vi "ADT681_Read.vi"(7 "Error In":errorcluster, 10 "DriverConnect in":T1={"InterfaceType"=enum."VISA", "OpenedSession"="COM4", "InterfaceSettings"={"Interface"=enum."RS232", "EOS 4 read"=enum."Default (=EOS 4 write)", "EOS 4 write"=enum."CR (\\r)", "TMO, ms"=2000, "Sett"=variant(cluster{"Baud Rate":u32, "Data Bits":u16, "Parity":u16, "Stop Bits":u16, "Flow Control":u16, "Eho":bool} {"Baud Rate"=75, "Data Bits"=0, "Parity"=0, "Stop Bits"=0, "Flow Control"=0, "Eho"=FALSE})}}) -> (0 "Error Out":errorcluster, 3 "DriverConnect out":T1={"InterfaceType"=enum."VISA", "OpenedSession"="COM4", "InterfaceSettings"={"Interface"=enum."RS232", "EOS 4 read"=enum."Default (=EOS 4 write)", "EOS 4 write"=enum."CR (\\r)", "TMO, ms"=2000, "Sett"=variant(cluster{"Baud Rate":u32, "Data Bits":u16, "Parity":u16, "Stop Bits":u16, "Flow Control":u16, "Eho":bool} {"Baud Rate"=75, "Data Bits"=0, "Parity"=0, "Stop Bits"=0, "Flow Control"=0, "Eho"=FALSE})}}, 4 "String":string)   [LabVIEW 2018]
uses:
  MOKO_LabViewLibrary/MokoLowLevel/MokoLowLovelControl/MLLC_ConnectCluster.ctl
  MOKO_LabViewLibrary/MokoLowLevel/MokoLowLovelControl/MLLC_InterfaceType.ctl
  MOKO_LabViewLibrary/MokoLowLevel/MokoLowLovelControl/MLLC_OpenedSession.ctl
  MOKO_LabViewLibrary/MokoLowLevel/MokoLowLovelControl/MLLC_InterfaceSettings.ctl
  MOKO_LabViewLibrary/MokoLowLevel/MokoLowLovelControl/MLLC_InterfaceKind.ctl
panel:
  out "read buffer":string
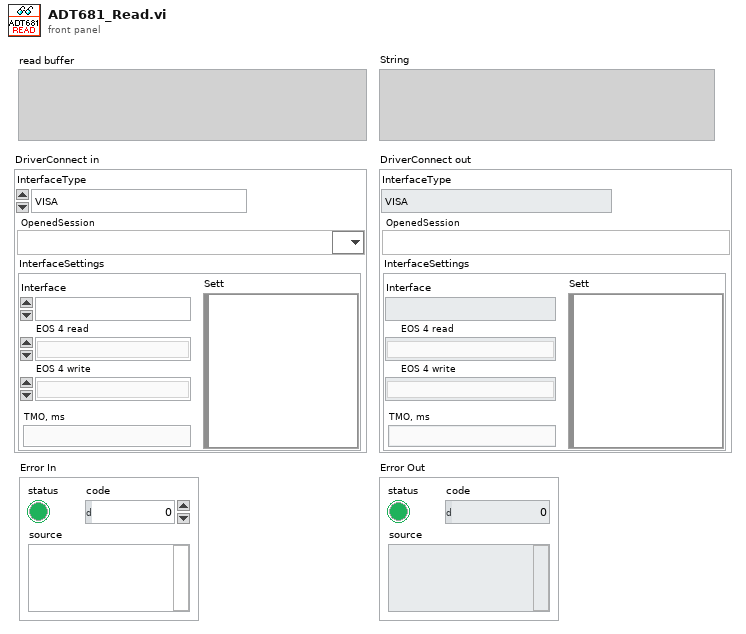
[diagram p1: front panel]
types:
  T1 = typedef "MLLC_ConnectCluster.ctl" = cluster{"InterfaceType":T2, "OpenedSession":T3, "InterfaceSettings":T4}
  T2 = typedef "MLLC_InterfaceType.ctl" = enum16{"VISA", "Prologix USB-GPIB"}
  T3 = typedef "MLLC_OpenedSession.ctl" = refnum<visa-resource-name>
  T4 = typedef "MLLC_InterfaceSettings.ctl" = cluster{"Interface":T5, "EOS 4 read":enum16{"Default (=EOS 4 write)", "CR (\\r)", "LF (\\n)", "None"}, "EOS 4 write":enum16{"CR+LF (\\r\\n)", "CR (\\r)", "LF (\\n)", "None"}, "TMO, ms":i32, "Sett":variant}
  T5 = typedef "MLLC_InterfaceKind.ctl" = enum16{"RS232", "GPIB", "USB", "Ethernet", "another"}
  T6 = enum16{"Default (=EOS 4 write)", "CR (\\r)", "LF (\\n)", "None"}
  T7 = enum16{"CR+LF (\\r\\n)", "CR (\\r)", "LF (\\n)", "None"}
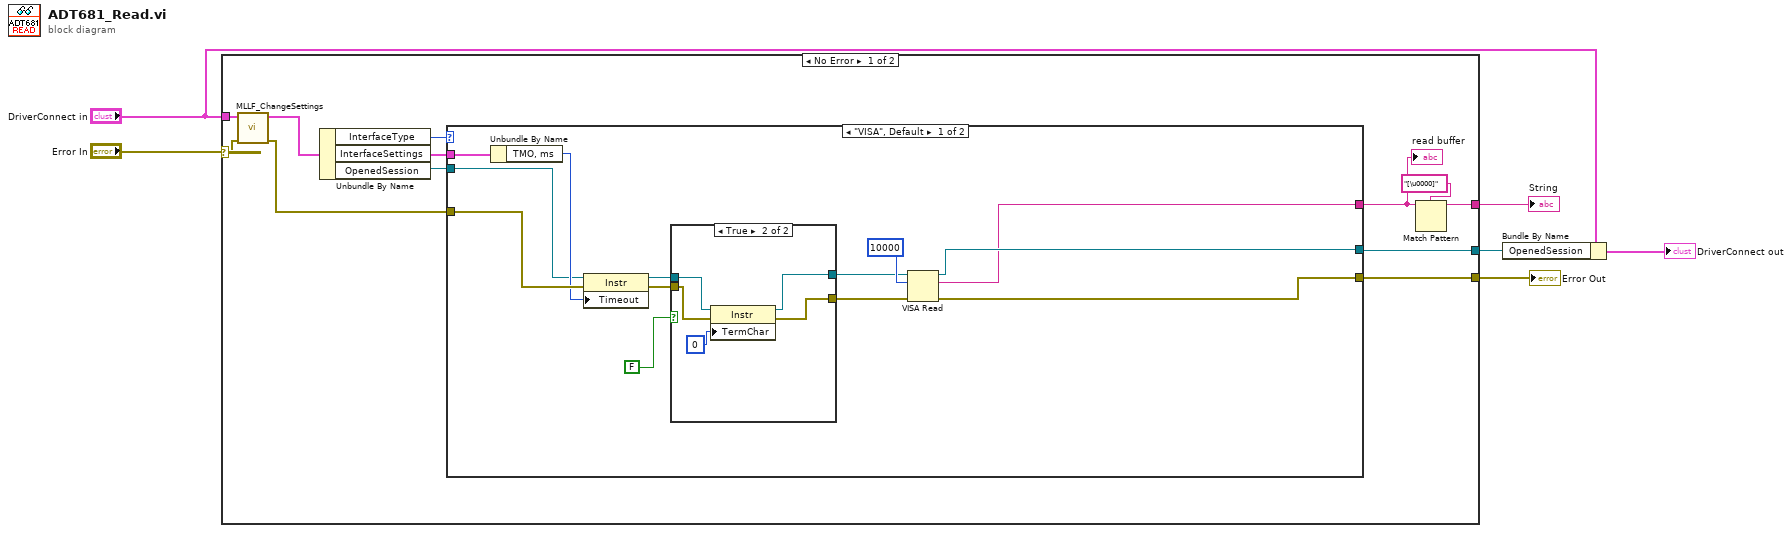
[diagram p0: block diagram]
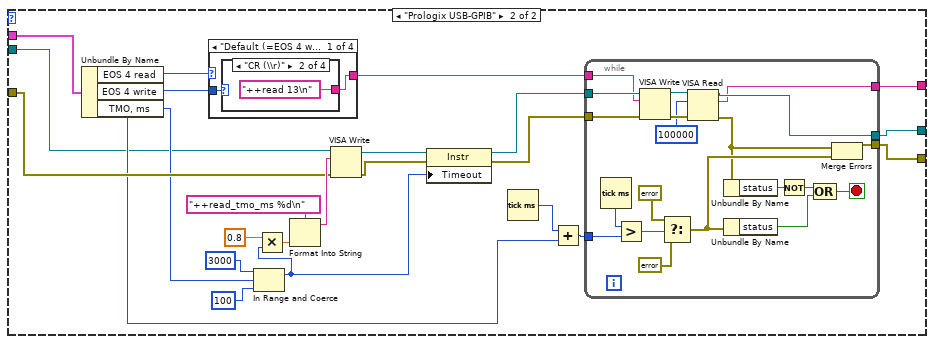
[diagram p3: hidden frame]
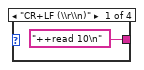
[diagram p4: hidden frame]
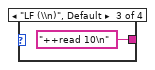
[diagram p5: hidden frame]
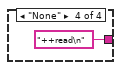
[diagram p6: hidden frame]
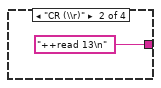
[diagram p7: hidden frame]
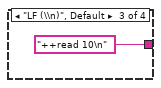
[diagram p8: hidden frame]
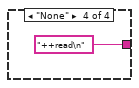
[diagram p9: hidden frame]
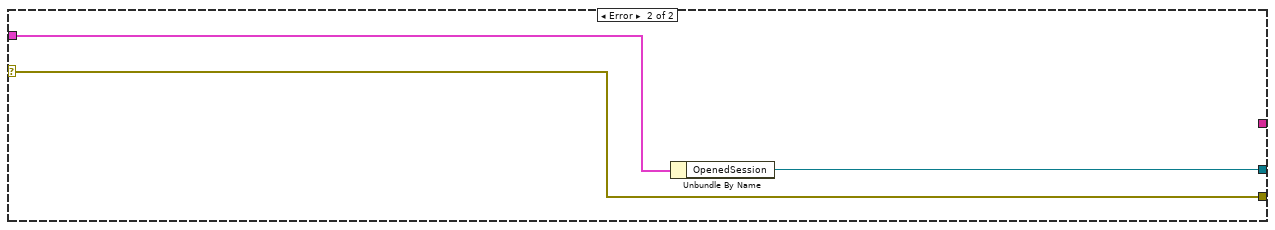
[diagram p10: hidden frame]
diagram:
  n1 = case shown="No Error" "Error In" {
    selector: "Error In" -> [w15 w93]
    tunnel: [w18 _] -> w6
    tunnel: [w17 w93] -> w4
    tunnel: [w16 w91] -> w2
    tunnel: "DriverConnect in" -> [w11 w92]
    frame No Error {
      n2 = call "MLLF_ChangeSettings.vi"("Error In"=w15, "DriverConnect in"=w11) -> ("Error Out"=w13:errorcluster, "DriverConnect out"=w10:T1)  [unwired: 4 in]
      n3 = Unbundle By Name(w10) -> ("InterfaceType"=w9:T2, "InterfaceSettings"=w8:T4, "OpenedSession"=w7:T3)
      n4 = case shown="\"VISA\", Default" w9 {
        tunnel: [w31 w44] -> w17
        tunnel: [w30 w43] -> w16
        tunnel: [w29 w61] -> w12
        tunnel: w13 -> [w28 w42]
        tunnel: w8 -> [w20 w60]
        tunnel: w7 -> [w19 w39]
        frame "VISA", Default {
          n5 = Unbundle By Name(w20) -> ("TMO, ms"=w27:i32)
          n6 = property class="Instr"(reference=w19, error in=w28, "Timeout"=w27) -> (reference out=w25:T3, error out=w24:errorcluster)
          n7 = case shown="True" FALSE {
            tunnel: w25 -> [w33 w37]
            tunnel: w24 -> [w32 w36]
            tunnel: [w33 w35] -> w23
            tunnel: [w32 w34] -> w22
            frame False {
            }
            frame True {
              n8 = property class="Instr"(reference=w37, error in=w36, "TermChar"=u8 0 ("Message Based Settings:Termination Character")) -> (reference out=w35:T3, error out=w34:errorcluster)
            }
          }
          n9 = VISA Read(VISA resource name=w23, byte count=u32 10000, error in (no error)=w22) -> (VISA resource name out=w30:T3, read buffer=w29:string, error out=w31:errorcluster)  [unwired: 1 out]
        }
        frame "Prologix USB-GPIB" {
          n10 = Unbundle By Name(w60) -> ("EOS 4 read"=w47:T6, "EOS 4 write"=w45:T7, "TMO, ms"=w41:i32)
          n11 = case shown="\"Default (=EOS 4 write)\"" w47 {
            tunnel: [w62 "++read 13\n" ("write buffer") "++read 10\n" ("write buffer") "++read\n" ("write buffer")] -> w46
            tunnel: w45 -> [w63 _ _ _]
            frame "Default (=EOS 4 write)" {
              n12 = case shown="\"CR (\\\\r)\"" w63 {
                tunnel: ["++read 10\n" ("write buffer") "++read 13\n" ("write buffer") "++read 10\n" ("write buffer") "++read\n" ("write buffer")] -> w62
                frame "CR+LF (\\r\\n)" {
                }
                frame "CR (\\r)" {
                }
                frame "LF (\\n)", Default {
                }
                frame "None" {
                }
              }
            }
            frame "CR (\\r)" {
            }
            frame "LF (\\n)", Default {
            }
            frame "None" {
            }
          }
          n13 = In Range and Coerce(upper limit=u32 3000, x=w41, lower limit=u32 100) -> (coerced(x)=w50:u32)  [unwired: 1 out]
          n14 = Multiply(x=0.8, y=w50) -> (x*y=w49:dbl)
          n15 = Format Into String(format string="++read_tmo_ms %d\n", w49) -> (resulting string=w51:string)  [unwired: 2 in, 1 out]
          n16 = VISA Write(VISA resource name=w39, write buffer=w51, error in (no error)=w42) -> (VISA resource name out=w59:T3, error out=w58:errorcluster)  [unwired: 1 out]
          n17 = property class="Instr"(reference=w59, error in=w58, "Timeout"=w50) -> (reference out=w56:T3, error out=w55:errorcluster)
          n18 = Tick Count (ms)() -> (millisecond timer value=w40:u32)
          n19 = Add(x=w40, y=w41) -> (x+y=w57:u32)
          n20 = while {
            tunnel: w55 -> [w81]
            tunnel: w56 -> [w82]
            tunnel: [w77] -> w43
            tunnel: [w90] -> w44
            tunnel: w57 -> [w88]
            tunnel: [w75] -> w61
            tunnel: w46 -> [w72]
            stop <- w85 stop-if-true
            n21 = Tick Count (ms)() -> (millisecond timer value=w89:u32)
            n22 = Greater?(x=w89, y=w88) -> (0:w87:bool)
            n23 = VISA Write(VISA resource name=w82, write buffer=w72, error in (no error)=w81) -> (VISA resource name out=w79:T3, error out=w80:errorcluster)  [unwired: 1 out]
            n24 = Select(t=errorcluster {"status"=TRUE, "code"=-1073807339, "source"="Prologix Read Timeout."} ("error in"), s=w87, f=errorcluster {"status"=FALSE, "code"=0, "source"=""} ("error in")) -> (s? t:f=w84:errorcluster)
            n25 = VISA Read(VISA resource name=w79, byte count=u32 100000, error in (no error)=w80) -> (VISA resource name out=w77:T3, read buffer=w75:string, error out=w76:errorcluster)  [unwired: 1 out]
            n26 = Unbundle By Name(w76) -> ("status"=w83:bool)
            n27 = Unbundle By Name(w84) -> ("status"=w73:bool)
            n28 = Not(x=w83) -> (.not. x?=w74:bool)
            n29 = Compound Arithmetic op=OR(w74, w73) -> (w85:bool)
            n30 = Merge Errors(w76, w84) -> (w90:errorcluster)
          }
        }
      }
      "read buffer" <- w12
      n31 = Match Pattern(string=w12, regular expression="[\u0000]") -> (before substring=w18:string)  [unwired: 1 in, 3 out]
    }
    frame Error {
      n32 = Unbundle By Name(w92) -> ("OpenedSession"=w91:T3)
    }
  }
  "String" <- w6
  "Error Out" <- w4
  n33 = Bundle By Name(cluster="DriverConnect in", "OpenedSession"=w2) -> (→"DriverConnect out":T1)
